vi "Format Data for Unicode-Import.vi"(11 "file (use dialog)":path=path "C:/Users/Jan-PhilippBrune/Desktop/My Unicode2.txt") -> (3 "subarray":string[][](array[string]))   [LabVIEW 2019, in "Language Editor.lvlib"]
uses:
  Language Editor.lvlib
panel:
  out "error out":errorcluster
  out "stripped path":path
  out "after substring":string
  out "appended array":string[][](array[string])
  # "Connector Pane"
  # "Locals"
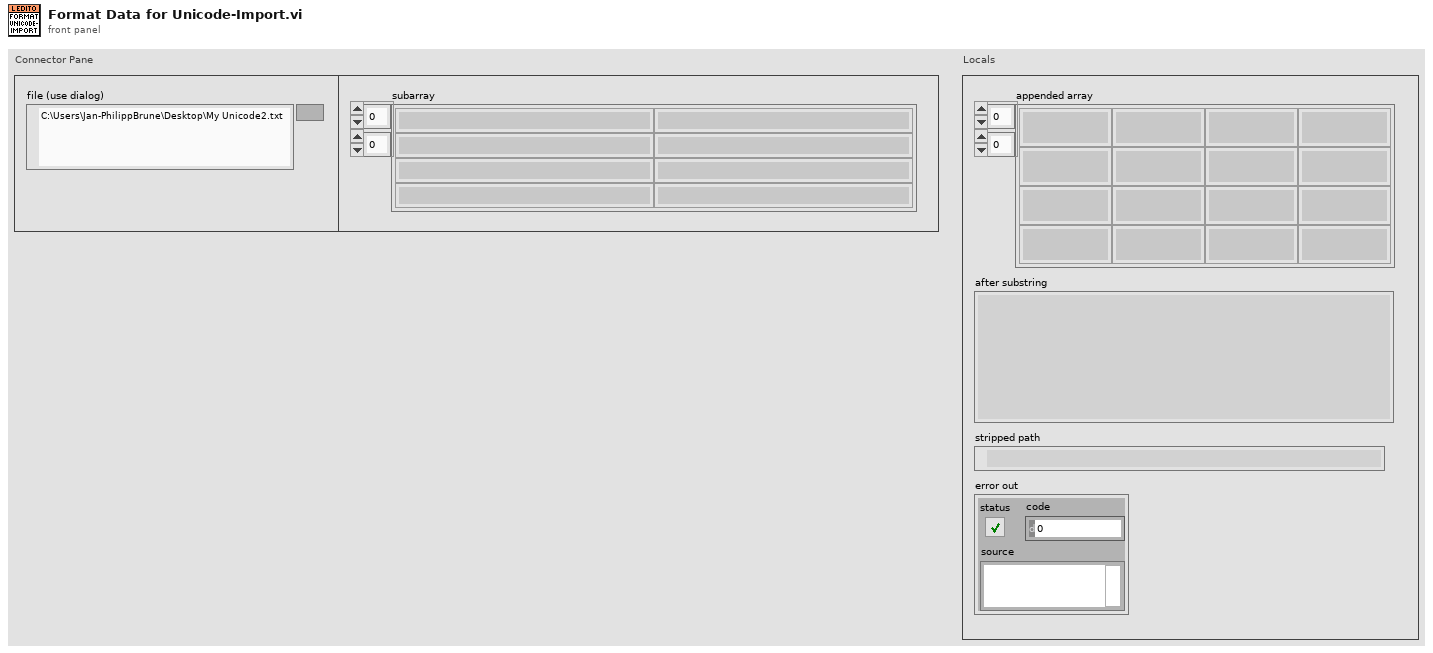
[diagram p1: front panel]
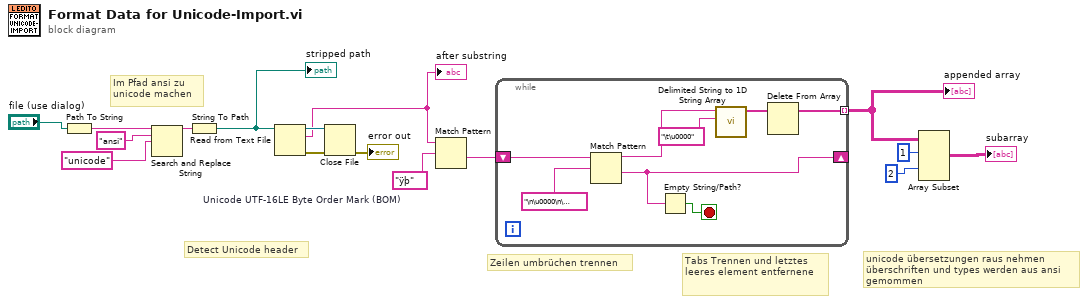
[diagram p0: block diagram]
diagram:
  w16 = "ÿþ"  # Unicode UTF-16LE Byte Order Mark (BOM)
  # "unicode übersetzungen raus nehmen\nüberschriften und types werden aus ansi\ngemommen"
  # "Tabs Trennen und letztes leeres element entfernene"
  # "Zeilen umbrüchen trennen"
  # "Im Pfad ansi zu\nunicode machen"
  # "Detect Unicode header"
  n1 = Path To String(path="file (use dialog)") -> (string=w8:string)
  n2 = Search and Replace String(input string=w8, search string="ansi", replace string="unicode" ("search string")) -> (result string=w5:string)  [unwired: 5 in, 3 out]
  n3 = String To Path(string=w5) -> (path=w3:path)
  "stripped path" <- w3
  n4 = Read from Text File(file (use dialog)=w3) -> (refnum out=w15:refnum<file>, text=w1:string, error out=w14:errorcluster)  [unwired: 3 in, 1 out]
  "after substring" <- w1
  n5 = Close File(refnum=w15, error in=w14) -> (error out=→"error out":errorcluster)  [unwired: 1 out]
  n6 = Match Pattern(string=w1, regular expression=w16) -> (after substring=w13:string)  [unwired: 1 in, 3 out]
  n7 = while {
    shift-right: [w22] -> _
    shift-left: w13 -> [w24]
    tunnel: [w17] -> w9 mode=indexing
    stop <- w21 stop-if-true
    n8 = Match Pattern(string=w24, regular expression="\n\u0000\n\u0000") -> (before substring=w20:string, after substring=w22:string)  [unwired: 1 in, 2 out]
    n9 = Empty String/Path?(string/path=w22) -> (empty?=w21:bool)
    n10 = call <vilib>:"Delimited String to 1D String Array.vi"("delimiter"="\t\u0000" ("regular expression"), "delimited string"=w20) -> ("string array"=w18:string[])  [unwired: 9 in]
    n11 = Delete From Array(array=w18) -> (array with subset deleted=w17:string[])  [unwired: 2 in, 1 out]
  }
  "appended array" <- w9
  n12 = Array Subset(array=w9, index (row)=1 ("index"), index (col)=2 ("index")) -> (→"subarray":string[][])  [unwired: 2 in]
